vi "Check Queue Priority Order.vi"() -> ()   [LabVIEW 2020]
doc: "Enqueue named classes with priority in reverse order to their priority\nTest if the Queue inspector returns them in priority order as expected"
uses:
  ActorFramework/Actor/Actor.lvclass
  ActorFramework/Message Enqueuer/Message Priority.ctl
  Test Harness/Priority/Low/Low.lvclass
  C:/Users/Neil/Documents/actor-framework/Core/ActorFramework/Message/Message.lvclass
  Test Harness/Priority/Normal/Normal.lvclass
  Test Harness/Priority/High/High.lvclass
  ActorFramework/Message Queue/Message Queue.lvclass/Message Queue.ctl
  ActorFramework/Message Enqueuer/Message Enqueuer.lvclass/Message Enqueuer.ctl
  ActorFramework/Stop Msg/Stop Msg.lvclass
  ActorFramework/Message Priority Queue/Priority Enqueue.vi
  <vilib>/addons/_JKI Toolkits/Caraya/classes/Assert/Assert Equal Value_Variant.vi
  <vilib>/addons/_JKI Toolkits/Caraya/classes/Test/Test.lvclass
  <vilib>/addons/_JKI Toolkits/Caraya/classes/Assert/Assert.lvclass
  ActorFramework/Message Queue/Message Queue.lvclass
  ActorFramework/Message Enqueuer/Message Enqueuer.lvclass
panel:
  out "Element Names":string[](array[string])
  out "# elements in queue":i32
  out "error out":errorcluster
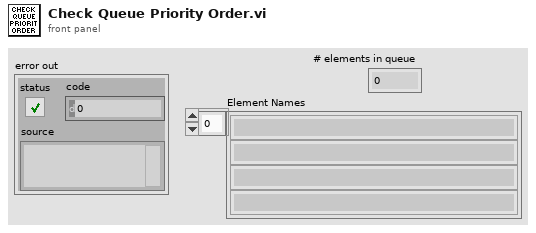
[diagram p1: front panel]
types:
  T1 = typedef "Actor Framework.lvlib/Message Enqueuer.lvclass/Message Priority.ctl" = enum16{"Low", "Normal", "High"}
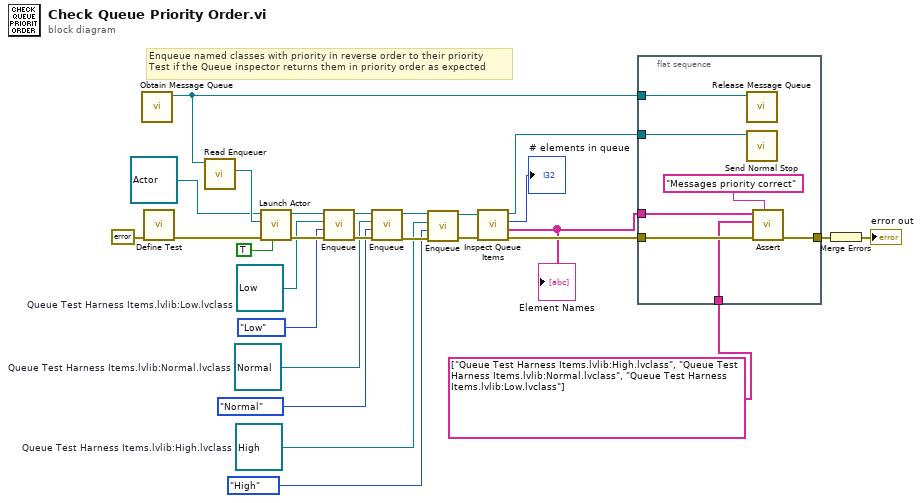
[diagram p0: block diagram]
diagram:
  w5 = refnum<class "High.lvclass"> refnum  # Queue Test Harness Items.lvlib:High.lvclass
  w7 = refnum<class "Normal.lvclass"> refnum  # Queue Test Harness Items.lvlib:Normal.lvclass
  w14 = refnum<class "Low.lvclass"> refnum  # Queue Test Harness Items.lvlib:Low.lvclass
  # "Enqueue named classes with priority in reverse order to their priority\nTest if the Queue inspector returns them in priority order as expected"
  n1 = call "Obtain Message Queue.vi"() -> ("Message Queue"=w22:refnum<class "Message Queue.lvclass">)  [unwired: 10 in, 1 out]
  n2 = call <vilib>:"Define Test.vi"("error in (no error)"=errorcluster {"status"=FALSE, "code"=0, "source"=""}) -> ("error out"=w25:errorcluster)  [unwired: 9 in, 1 out]
  n3 = call "Read Enqueuer.vi"("Message Queue"=w22) -> ("Message Enqueuer"=w24:refnum<class "Message Enqueuer.lvclass">)  [unwired: 10 in]
  n4 = call "Launch Actor.vi"("Open Actor Core front panel? (F)"=TRUE, "error in (no error)"=w25, "Actor-to-Caller Enqueuer"=w24, "Actor"=refnum<class "Actor.lvclass"> refnum) -> ("error out"=w18:errorcluster, "Caller-To-Actor Enqueuer"=w19:refnum<class "Message Enqueuer.lvclass">)  [unwired: 6 in]
  n5 = call "Enqueue.vi"("error in (no error)"=w18, "Message Priority (Normal)"=Message_Priority."Low", "Message"=w14, "Message Enqueuer in"=w19) -> ("error out"=w8:errorcluster, "Message Enqueuer out"=w13:refnum<class "Message Enqueuer.lvclass">)  [unwired: 6 in]
  n6 = call "Enqueue.vi"("error in (no error)"=w8, "Message Priority (Normal)"=Message_Priority."Normal", "Message"=w7, "Message Enqueuer in"=w13) -> ("error out"=w9:errorcluster, "Message Enqueuer out"=w12:refnum<class "Message Enqueuer.lvclass">)  [unwired: 6 in]
  n7 = call "Enqueue.vi"("error in (no error)"=w9, "Message Priority (Normal)"=Message_Priority."High", "Message"=w5, "Message Enqueuer in"=w12) -> ("error out"=w10:errorcluster, "Message Enqueuer out"=w11:refnum<class "Message Enqueuer.lvclass">)  [unwired: 6 in]
  n8 = call "Inspect Queue Items.vi"("error in (no error)"=w10, "Message Enqueuer in"=w11) -> ("error out"=w16:errorcluster, "Element Names"=w3:string[], "# elements in queue"=→"# elements in queue":i32, "Message Enqueuer out"=w17:refnum<class "Message Enqueuer.lvclass">)  [unwired: 6 in]
  "Element Names" <- w3
  n9 = flat-sequence {
    tunnel: [w33] -> w27
    tunnel: w16 -> [w32]
    tunnel: w22 -> [w31]
    tunnel: w17 -> [w30]
    tunnel: w3 -> [w29]
    tunnel: string[] ["Queue Test Harness Items.lvlib:High.lvclass", "Queue Test Harness Items.lvlib:Normal.lvclass", "Queue Test Harness Items.lvlib:Low.lvclass"] ("Element Names") -> [w28]
    frame #0 {
      n10 = call "Release Message Queue.vi"("Message Queue"=w31) -> ()  [unwired: 9 in, 2 out]
      n11 = call "Send Normal Stop.vi"("Message Enqueuer"=w30) -> ()  [unwired: 10 in, 1 out]
      n12 = call-poly <vilib>:"Assert.vi"("Label"="Messages priority correct" ("Label (VI Title)"), "error in (no error)"=w32, "Actual"=w28, "Expected"=w29) -> ("error out"=w33:errorcluster)  [unwired: 6 in, 1 out]
    }
  }
  n13 = Merge Errors(w27) -> (→"error out":errorcluster)
